vi "Prepare DAQmx Module.vi"(4 "Create Scaling (F)":bool, 6 "On Demand (F)":bool, 8 "error in (no error)":errorcluster, 11 "Module in":refnum<class "Module.lvclass">) -> (0 "error out":errorcluster, 1 "Scaling":refnum<class "Scaling.lvclass">, 2 "Group":refnum<class "Group DBL.lvclass">, 3 "Module out":refnum<class "Module.lvclass">, 5 "DAQmx Task":refnum<k21>, 7 "Sampling Config":T1)   [LabVIEW 2020, in "VolatusDAQ.lvlib"]
uses:
  VolatusDAQ.lvlib
  Volatus/Module/Module.lvclass
  lv-vecto/Vecto/Group DBL/Group DBL.lvclass
  C:/dev/lv20CE/relink/lv-vecto/Vecto/Group/Group.lvclass
  VolatusDAQConfig/Sampling Config.ctl
  VolatusData/Scaling/Scaling.lvclass
  Volatus/Event Level.ctl
  Volatus/Module/Module.lvclass/Module.ctl
  VolatusConfig/VolatusConfigElement/VolatusConfigElement.lvclass/VolatusConfigElement.ctl
  Volatus/Module/Config.vi
  VolatusConfig/VolatusConfigElement/Element.vi
  VolatusConfig/Channel/Channel Config.lvclass
  C:/dev/lv20CE/relink/lv-volatus/VolatusConfig/VolatusConfigElement/VolatusConfigElement.lvclass
  VolatusConfig/Group/Group Config.lvclass
  VolatusConfig/Scaling/Create (Group).vi
  VolatusData/Scaling/Create (Config).vi
  VolatusConfig/Task/Task Config.lvclass
  <vilib>/DAQmx/configure/timing.llb/DAQmx Timing (Sample Clock).vi
  VolatusDAQConfig/DAQmxChannel/DAQmxChannel.lvclass
  VolatusDAQConfig/VolatusDAQConfig.lvlib
  Volatus/Volatus.lvlib
  VolatusConfig/VolatusConfigElement/VolatusConfigElement.lvclass
  C:/dev/lv20CE/relink/lv-volatus/VolatusConfig/Channel/Channel Config.lvclass
  C:/dev/lv20CE/relink/lv-vecto/Vecto/Group DBL/Group DBL.lvclass
  C:/dev/lv20CE/relink/lv-volatus/VolatusConfig/Group/Group Config.lvclass
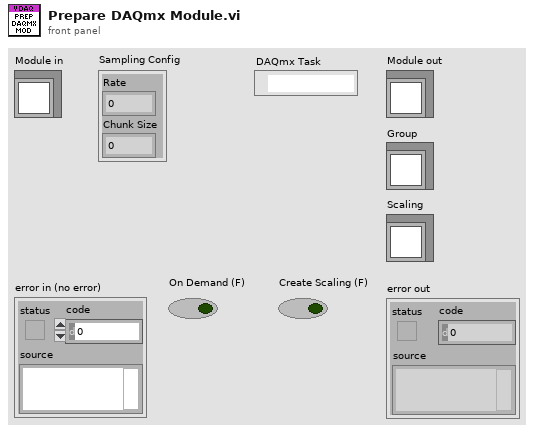
[diagram p1: front panel]
types:
  T1 = typedef "VolatusDAQConfig.lvlib/Sampling Config.ctl" = cluster{"Rate":dbl, "Chunk Size":i32}
  T2 = typedef "Volatus.lvlib/Event Level.ctl" = enum16{"Debug", "Info", "Warning", "Error"}
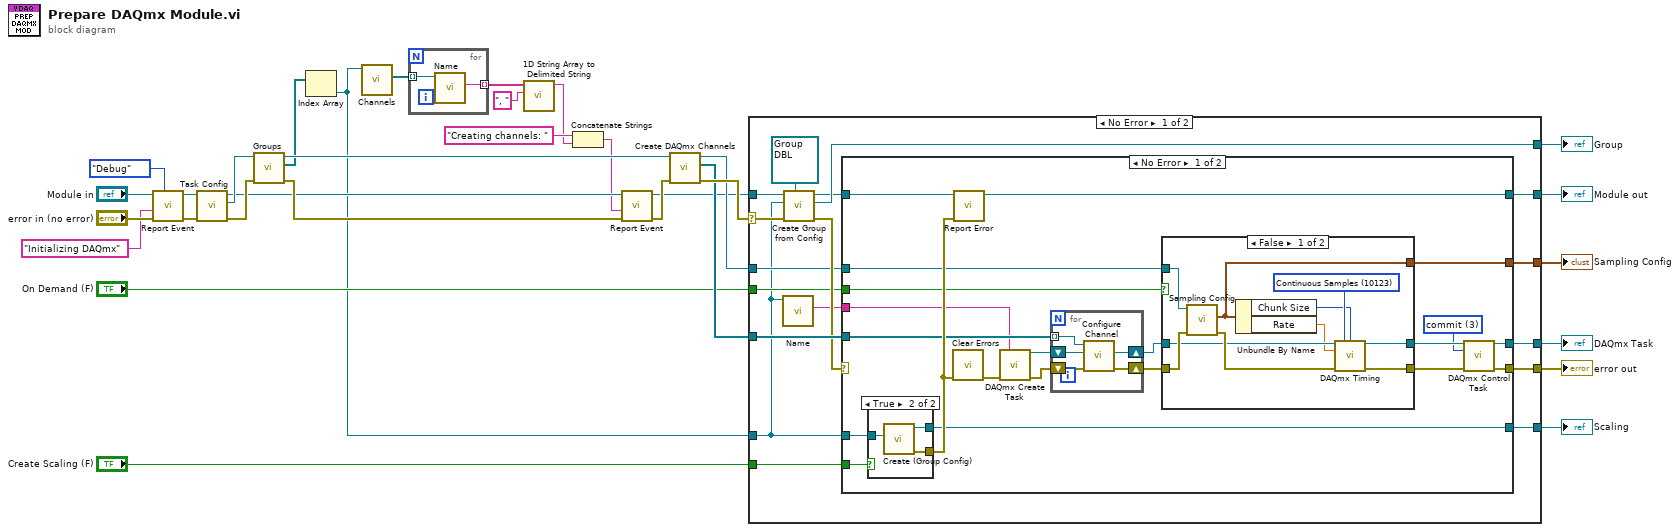
[diagram p0: block diagram]
diagram:
  n1 = call "Report Event.vi"("Level (Info)"=Event_Level."Debug", "error in (no error)"="error in (no error)", "Message"="Initializing DAQmx", "Module in"="Module in") -> ("error out"=w12:errorcluster, "Module out"=w10:refnum<class "Module.lvclass">)  [unwired: 6 in]
  n2 = call "Task Config.vi"("error in (no error)"=w12, "Module in"=w10) -> ("error out"=w29:errorcluster, "Task Config"=w28:refnum<class "Task Config.lvclass">, "Module out"=w25:refnum<class "Module.lvclass">)  [unwired: 7 in]
  n3 = call "Groups.vi"("error in (no error)"=w29, "Task in"=w28) -> ("error out"=w32:errorcluster, "Groups"=w26:refnum<class "Group Config.lvclass">[], "Task out"=w27:refnum<class "Task Config.lvclass">)  [unwired: 7 in]
  n4 = Index Array(array=w26) -> (element=w13:refnum<class "Group Config.lvclass">)  [unwired: 1 in]
  n5 = call "Channels.vi"("Group in"=w13) -> ("Channels"=w7:refnum<class "Channel Config.lvclass">[])  [unwired: 8 in, 2 out]
  n6 = for {
    tunnel: w7 -> [w34] mode=indexing
    tunnel: [w33] -> w6 mode=indexing
    n7 = call "Name.vi"("VolatusConfigElement in"=w34) -> ("Name"=w33:string)  [unwired: 8 in, 2 out]
  }
  n8 = call <vilib>:"1D String Array to Delimited String.vi"("delimiter"=", ", "string array"=w6) -> ("delimited string"=w2:string)  [unwired: 9 in]
  n9 = Concatenate Strings("Creating channels: " ("Message"), w2) -> (w1:string)
  n10 = call "Report Event.vi"("error in (no error)"=w32, "Message"=w1, "Module in"=w25) -> ("error out"=w31:errorcluster, "Module out"=w4:refnum<class "Module.lvclass">)  [unwired: 7 in]
  n11 = call "Create DAQmx Channels.vi"("error in (no error)"=w31, "Task In"=w27) -> ("error out"=w30:errorcluster, "DAQmxChannels"=w22:refnum<class "DAQmxChannel.lvclass">[], "Task"=w14:refnum<class "Task Config.lvclass">)  [unwired: 7 in]
  n12 = case shown="No Error" w30 {
    selector: w30 -> [w51 w95]
    tunnel: w4 -> [w50 w96]
    tunnel: [w48 _] -> w23
    tunnel: w22 -> [w47 _]
    tunnel: [w46 _] -> w21
    tunnel: [w35 w96] -> w20
    tunnel: [w45 w95] -> w19
    tunnel: [w44 _] -> w18
    tunnel: "Create Scaling (F)" -> [w43 _]
    tunnel: "On Demand (F)" -> [w41 _]
    tunnel: [w40 _] -> w15
    tunnel: w14 -> [w39 _]
    tunnel: w13 -> [w38 _]
    frame No Error {
      n13 = call "Name.vi"("VolatusConfigElement in"=w38) -> ("Name"=w37:string)  [unwired: 8 in, 2 out]
      n14 = call "Create Group from Config.vi"("Group Type (Abstract)"=refnum<class "Group DBL.lvclass"> refnum ("Vecto.lvlib:Group.lvclass"), "error in (no error)"=w51, "Group Config"=w38, "Module in"=w50) -> ("error out"=w42:errorcluster, "Group"=w48:refnum<class "Group DBL.lvclass">, "Module out"=w36:refnum<class "Module.lvclass">)  [unwired: 5 in]
      n15 = case shown="No Error" w42 {
        selector: w42 -> [_ w94]
        tunnel: w47 -> [w66 _]
        tunnel: [w65 _] -> w46
        tunnel: [w64 w94] -> w45
        tunnel: w38 -> [w63 _]
        tunnel: [w62 _] -> w44
        tunnel: w43 -> [w61 _]
        tunnel: w41 -> [w60 _]
        tunnel: [w59 _] -> w40
        tunnel: w39 -> [w58 _]
        tunnel: w37 -> [w56 _]
        tunnel: w36 -> [w54 w93]
        tunnel: [w52 w93] -> w35
        frame No Error {
          w67 = 3 items=["verify"=2, "reserve"=4, "commit"=3, "unreserve"=5, "abort"=6] ("action")
          n16 = case shown="True" w61 {
            tunnel: w63 -> [_ w75]
            tunnel: [_ w74] -> w62
            tunnel: [_ w73] -> w72
            frame False {
            }
            frame True {
              n17 = call "Create (Group Config).vi"("Group Config"=w75) -> ("error out"=w73:errorcluster, "Scaling out"=w74:refnum<class "Scaling.lvclass">)  [unwired: 9 in]
            }
          }
          n18 = call <vilib>:"Clear Errors.vi"("error in (no error)"=w72) -> ("error out"=w53:errorcluster)  [unwired: 5 in, 1 out]
          n19 = call "Report Error.vi"("error in (no error)"=w72, "Module in"=w54) -> ("Module out"=w52:refnum<class "Module.lvclass">)  [unwired: 8 in, 1 out]
          n20 = call <vilib>:"DAQmx Create Task.vi"("new task name"=w56, "error in"=w53) -> ("task out"=w57:refnum<k21>, "error out"=w55:errorcluster)  [unwired: 12 in]
          n21 = for {
            shift-right: [w78] -> w70
            shift-left: w57 -> [w79]
            tunnel: w66 -> [w80] mode=indexing
            shift-right: [w76] -> w71
            shift-left: w55 -> [w77]
            n22 = call-dynamic "Configure Channel.vi"("error in (no error)"=w77, "DAQmx Task In"=w79, "DAQmxChannel in"=w80) -> ("error out"=w76:errorcluster, "DAQmx Task"=w78:refnum<k21>)  [unwired: 7 in]
          }
          n23 = case shown="False" w60 {
            tunnel: w71 -> [w89 w91]
            tunnel: w70 -> [w88 w92]
            tunnel: [w86 w91] -> w69
            tunnel: [w85 w92] -> w68
            tunnel: [w82 _] -> w59
            tunnel: w58 -> [w81 _]
            frame False {
              w87 = 10123 items=["Finite Samples"=10178, "Continuous Samples"=10123, "Hardware Timed Single Point"=12522] ("sample mode")
              n24 = call "Sampling Config.vi"("error in (no error)"=w89, "Task In"=w81) -> ("error out"=w90:errorcluster, "Sampling Config"=w82:T1)  [unwired: 7 in, 1 out]
              n25 = Unbundle By Name(w82) -> ("Chunk Size"=w83:i32, "Rate"=w84:dbl)
              n26 = call-poly <vilib>:"DAQmx Timing.vi"("task/channels in"=w88, "sample mode"=w87, "samples per channel"=w83, "rate"=w84, "error in"=w90) -> ("task out"=w85:refnum<k21>, "error out"=w86:errorcluster)  [unwired: 9 in]
            }
            frame True {
            }
          }
          n27 = call <vilib>:"DAQmx Control Task.vi"("task/channels in"=w68, "action"=w67, "error in"=w69) -> ("task out"=w65:refnum<k21>, "error out"=w64:errorcluster)  [unwired: 11 in]
        }
        frame Error {
        }
      }
    }
    frame Error {
    }
  }
  "Module out" <- w20
  "error out" <- w19
  "Group" <- w23
  "DAQmx Task" <- w21
  "Sampling Config" <- w15
  "Scaling" <- w18
